vi "RemoteVI Set Modifier Keys.vi"(0 "mods":u8, 11 "error in":errorcluster) -> (15 "error out":errorcluster)   [LabVIEW 2020, in "RemoteVI.lvlib"]
doc: "Makes the key state of LabVIEW's UI thread show the modifier keys mods as held (1 Shift, 2 Ctrl, 4 Alt - see RemoteVI Track Modifiers.vi) and all others of the three as released. LabVIEW reads the modifiers of every mouse and key event with GetKeyState, and a POSTED message does not update that state - only real input does (measured: a posted Shift-click arrived without Shift). So the state is written directly: user32 GetKeyboardState.vi and user32 SetKeyboardState.vi, both configured to run in LabVIEW's UI thread, because a thread's key state can only be read and written by that thread. For each modifier bit 0x80 of the generic and the left key (VK_SHIFT 0x10 + VK_LSHIFT 0xA0, VK_CONTROL 0x11 + VK_LCONTROL 0xA2, VK_MENU 0x12 + VK_LMENU 0xA4) is set or cleared, the right key (0xA1, 0xA3, 0xA5) is cleared; the toggle bit 0x01 and every other key are kept. Only that thread's state changes: the host's keyboard, GetAsyncKeyState and other programs are untouched, and the next real input LabVIEW receives replaces it. Do NOT call it while a LabVIEW popup is open: its modal loop holds the UI thread (RemoteVI Service Client.vi checks). An incoming error skips the work."
uses:
  RemoteVI.lvlib
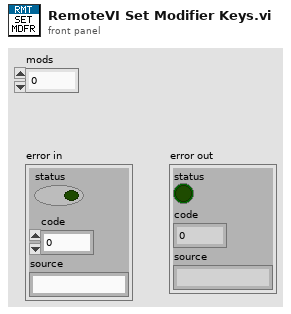
[diagram p1: front panel]
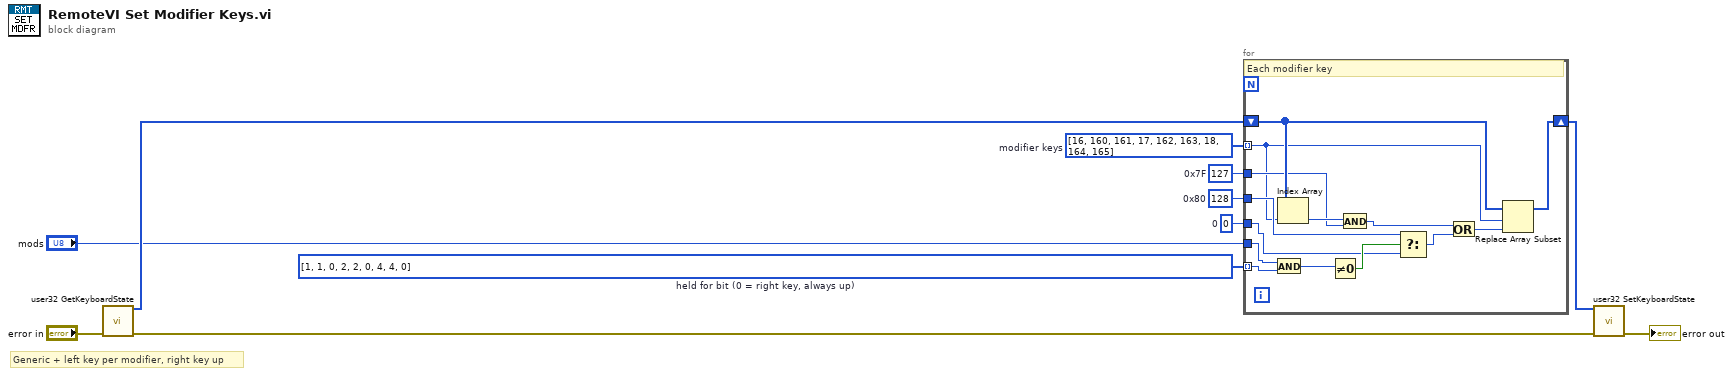
[diagram p0: block diagram]
diagram:
  w7 = u8 0  # 0
  w6 = u8 128  # 0x80
  w5 = u8 127  # 0x7F
  w4 = u8[] [1, 1, 0, 2, 2, 0, 4, 4, 0]  # held for bit (0 = right key, always up)
  w3 = i32[] [16, 160, 161, 17, 162, 163, 18, 164, 165]  # modifier keys
  # "Generic + left key per modifier, right key up"
  n1 = call "user32 GetKeyboardState.vi"("error in"="error in") -> ("key state"=w8:u8[], "error out"=w9:errorcluster)  [unwired: 12 in, 1 out]
  n2 = for {
    tunnel: w3 -> [w12] mode=indexing
    tunnel: w4 -> [w13] mode=indexing
    tunnel: "mods" -> [w14]
    tunnel: w5 -> [w15]
    tunnel: w6 -> [w16]
    tunnel: w7 -> [w17]
    shift-right: [w19] -> w10
    shift-left: w8 -> [w18]
    # "Each modifier key"
    n3 = And(x=w14, y=w13) -> (x .and. y?=w22:u8)
    n4 = Index Array(array=w18, index=w12) -> (element=w20:u8)
    n5 = Not Equal To 0?(x=w22) -> (x != 0?=w23:bool)
    n6 = And(x=w20, y=w15) -> (x .and. y?=w21:u8)
    n7 = Select(t=w16, s=w23, f=w17) -> (s? t:f=w24:u8)
    n8 = Or(x=w21, y=w24) -> (x .or. y?=w25:u8)
    n9 = Replace Array Subset(array=w18, new element=w25, index=w12) -> (w19:u8[])
  }
  n10 = call "user32 SetKeyboardState.vi"("key state"=w10, "error in"=w9) -> ("error out"=→"error out":errorcluster)  [unwired: 12 in, 1 out]
